vi "NLTest_init.vi"(8 "error in (no error)":errorcluster) -> (0 "error out":errorcluster, 3 "NLTest out":refnum<class "NLTest.lvclass">)   [LabVIEW 2017, in "NLTest.lvclass"]
uses:
  NLTest.lvclass
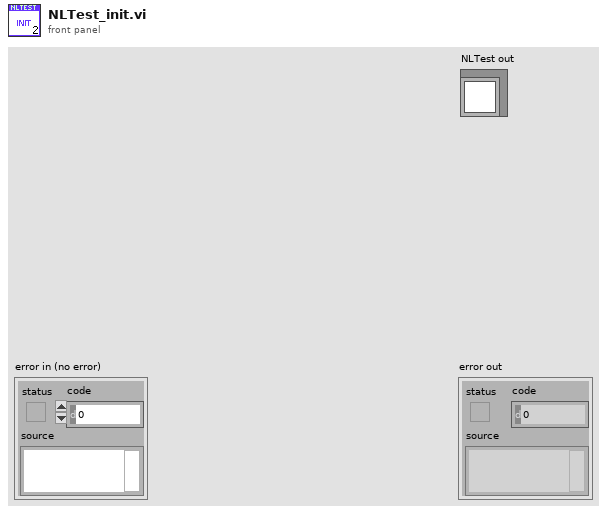
[diagram p1: front panel]
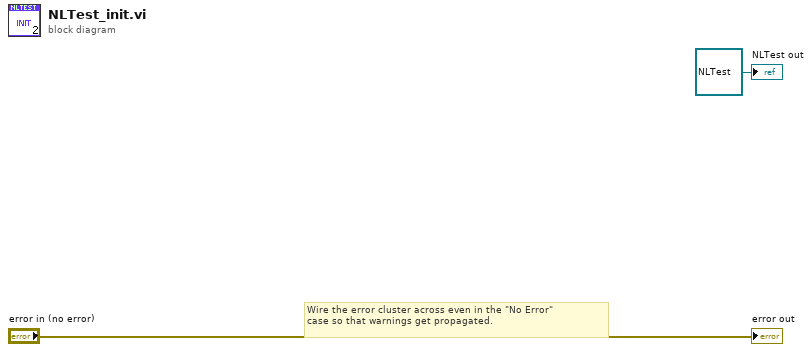
[diagram p0: block diagram]
diagram:
  # "Wire the error cluster across even in the \"No Error\"\ncase so that warnings get propagated."
  "error out" <- "error in (no error)"
  "NLTest out" <- refnum<class "NLTest.lvclass"> refnum ("NLTest out")
